vi "Init.vi"(8 "error in (no error)":errorcluster caption="错误输入（无错误）", 10 "procotol_path":path, 11 "Procotol_class 输入":refnum<class "Procotol_class.lvclass">) -> (0 "error out":errorcluster caption="错误输出", 3 "Procotol_class 输出":refnum<class "Procotol_class.lvclass">)   [LabVIEW 2025, in "Procotol_class.lvclass"]
uses:
  Procotol_class.lvclass
  ID_arr.ctl
  Procotol_class.lvclass/Procotol_class.ctl
panel:
  in  "组合框":T1
  # "这个协议的路径建议你使用\n路径管理类传入路径"
  # "这个类labview2017不支持\n动态传引用\n啊啊啊啊啊啊啊"
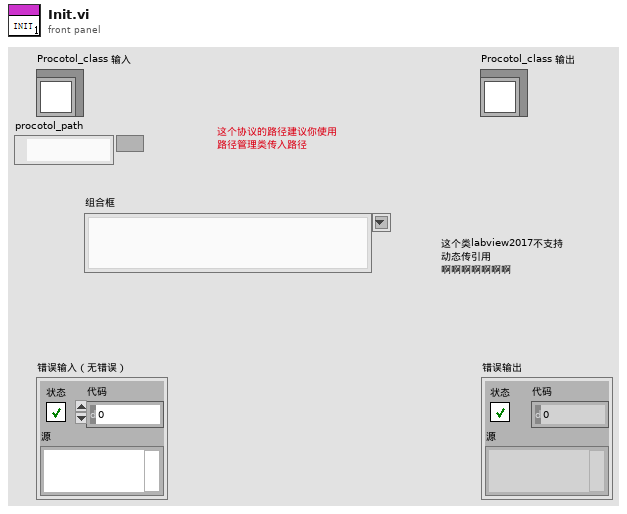
[diagram p1: front panel]
types:
  T1 = typedef "Procotol_class.lvclass/ID_arr.ctl" = string
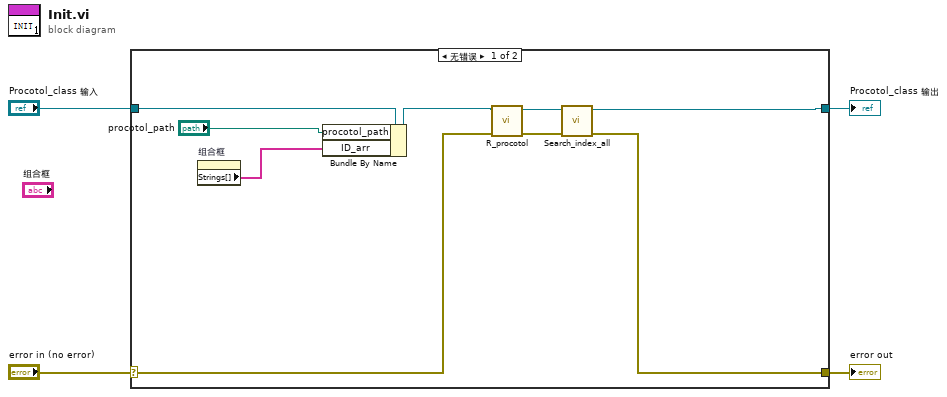
[diagram p0: block diagram]
diagram:
  n1 = case shown="无错误" "error in (no error)" {
    selector: "error in (no error)" -> [w10 w15]
    tunnel: [w6 w15] -> w3
    tunnel: [w7 w14] -> w1
    tunnel: "Procotol_class 输入" -> [w13 w14]
    frame No Error {
      n2 = property on="组合框" class="CmbBox (严格)"() -> ("Strings[]"=w5:string[])  [unwired: 2 in, 2 out]
      n3 = Bundle By Name(cluster=w13, "procotol_path"="procotol_path", "ID_arr"=w5) -> (w11:refnum<class "Procotol_class.lvclass">)
      n4 = call-dynamic "R_procotol.vi"("error in (no error)"=w10, "Procotol_class 输入"=w11) -> ("error out"=w8:errorcluster, "Procotol_class 输出"=w9:refnum<class "Procotol_class.lvclass">)  [unwired: 8 in]
      n5 = call-dynamic "Search_index_all.vi"("error in (no error)"=w8, "Procotol_class 输入"=w9) -> ("error out"=w6:errorcluster, "Procotol_class 输出"=w7:refnum<class "Procotol_class.lvclass">)  [unwired: 8 in]
    }
    frame Error {
    }
  }
  "error out" <- w3
  "Procotol_class 输出" <- w1
